vi "LoadSystemDefinition.vi"(8 "error in (no error)":errorcluster, 11 "SysDef.Path":path) -> (0 "error out":errorcluster, 2 "Aliases.Outputs":T1[](array[typedef]), 3 "Aliases.All":T1[](array[typedef]))   [LabVIEW 2015, in "Simple Sequence Tools - Editor.lvlib"]
uses:
  Simple Sequence Tools - Editor.lvlib
  Shared/Types/Channel.Properties.ctl
  NationalInstruments.VeriStand.SystemStorage
  NationalInstruments.VeriStand.SystemDefinitionAPI
  Shared/Simple Sequence Tools - Shared.lvlib
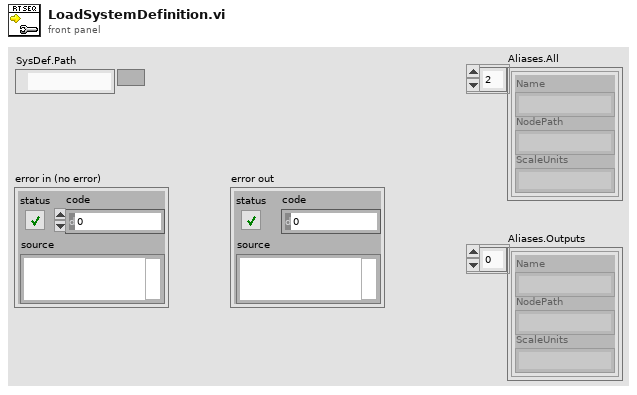
[diagram p1: front panel]
types:
  T1 = typedef "Simple Sequence Tools - Shared.lvlib/Channel.Properties.ctl" = cluster{"Name":string, "NodePath":string, "ScaleUnits":string}
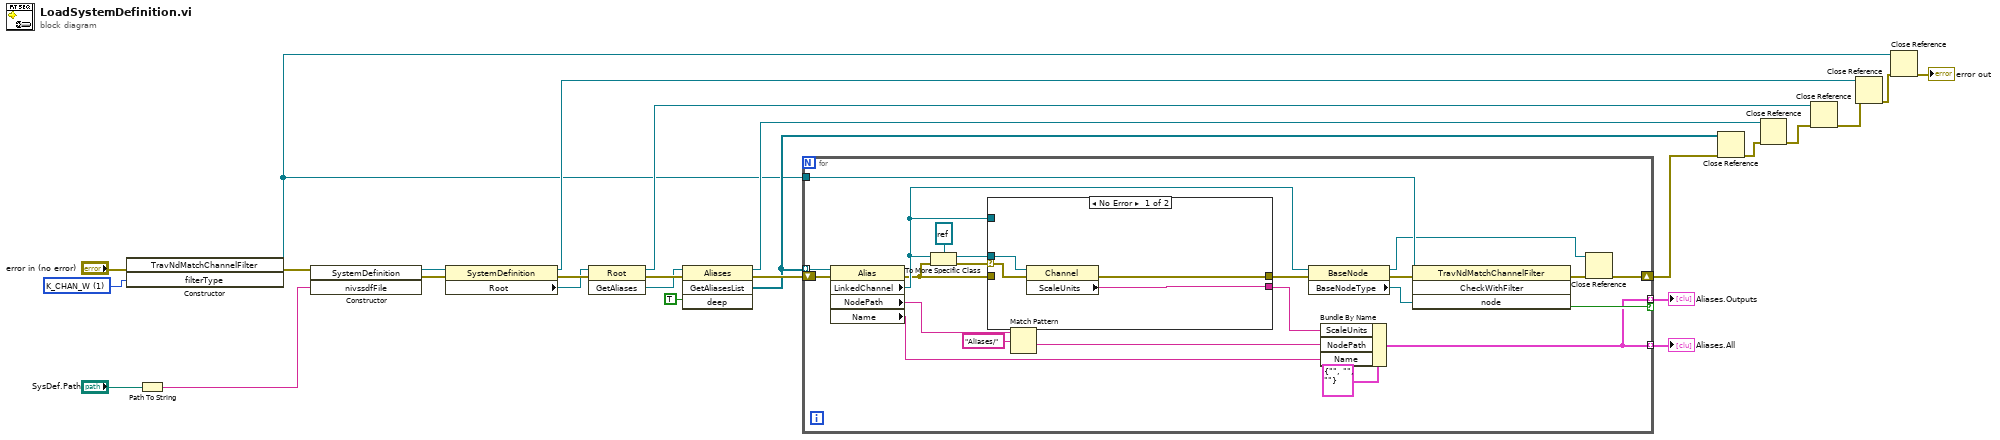
[diagram p0: block diagram]
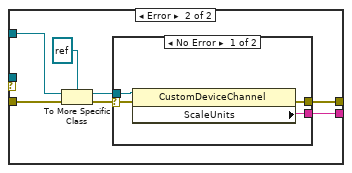
[diagram p2: hidden frame]
diagram:
  w16 = u8 1 items=["K_CHAN_R", "K_CHAN_W", "K_CHAN_VOLT", "K_CHAN_FAULT"] ("filterType")
  n1 = constructor class="TravNdMatchChannelFilter"(error in="error in (no error)", "filterType"=w16) -> (reference out=w9:refnum<k24>, error out=w14:errorcluster)  [unwired: 2 in, 2 out]
  n2 = Path To String(path="SysDef.Path") -> (string=w19:string)
  n3 = constructor class="SystemDefinition"(error in=w14, "nivssdfFile"=w19) -> (reference out=w20:refnum<k24>, error out=w25:errorcluster)  [unwired: 2 in, 2 out]
  n4 = property class="SystemDefinition"(reference=w20, error in=w25) -> (reference out=w13:refnum<k24>, error out=w24:errorcluster, "Root"=w21:refnum<k24>)
  n5 = invoke class="Root" method="GetAliases"(reference=w21, error in=w24) -> (reference out=w12:refnum<k24>, error out=w23:errorcluster, "GetAliases"=w17:refnum<k24>)  [unwired: 1 in]
  n6 = invoke class="Aliases" method="GetAliasesList"(reference=w17, error in=w23, "deep"=TRUE) -> (reference out=w11:refnum<k24>, error out=w26:errorcluster, "GetAliasesList"=w10:refnum<k24>[])  [unwired: 1 in, 1 out]
  n7 = for {
    tunnel: w10 -> [w48] mode=indexing
    tunnel: [w30] -> w2 mode=indexing if=w46
    shift-right: [w42] -> w4
    shift-left: w26 -> [w47]
    tunnel: [w30] -> w1 mode=indexing
    tunnel: w9 -> [w44]
    n8 = property class="Alias"(reference=w48, error in=w47) -> (error out=w37:errorcluster, "LinkedChannel"=w38:refnum<k24>, "NodePath"=w29:string, "Name"=w33:string)  [unwired: 1 out]
    n9 = To More Specific Class(target class=refnum<k24> refnum ("new reference"), reference=w38, error in=w37) -> (specific class reference=w40:refnum<k24>, error out=w41:errorcluster)
    n10 = case shown="No Error" w41 {
      selector: w41 -> [w51 _]
      tunnel: w40 -> [w52 _]
      tunnel: [w49 w54] -> w36
      tunnel: w38 -> [_ w59]
      tunnel: w37 -> [_ w58]
      tunnel: [w50 w53] -> w31
      frame No Error {
        n11 = property class="Channel"(reference=w52, error in=w51) -> (error out=w49:errorcluster, "ScaleUnits"=w50:string)  [unwired: 1 out]
      }
      frame Error {
        n12 = To More Specific Class(target class=refnum<k24> refnum ("new reference"), reference=w59, error in=w58) -> (specific class reference=w56:refnum<k24>, error out=w55:errorcluster)
        n13 = case shown="No Error" w55 {
          selector: w55 -> [w62 _]
          tunnel: w56 -> [w63 _]
          tunnel: [w61 _] -> w54
          tunnel: [w60 _] -> w53
          frame No Error {
            n14 = property class="CustomDeviceChannel"(reference=w63, error in=w62) -> (error out=w61:errorcluster, "ScaleUnits"=w60:string)  [unwired: 1 out]
          }
          frame Error {
          }
        }
      }
    }
    n15 = Match Pattern(string=w29, regular expression="Aliases/") -> (after substring=w28:string)  [unwired: 1 in, 3 out]
    n16 = property class="BaseNode"(reference=w38, error in=w36) -> (reference out=w35:refnum<k24>, error out=w45:errorcluster, "BaseNodeType"=w43:refnum<k24>)
    n17 = Bundle By Name(cluster=T1 {"Name"="", "NodePath"="", "ScaleUnits"=""}, "ScaleUnits"=w31, "NodePath"=w28, "Name"=w33) -> (w30:T1)
    n18 = invoke class="TravNdMatchChannelFilter" method="CheckWithFilter"(reference=w44, error in=w45, "node"=w43) -> (error out=w34:errorcluster, "CheckWithFilter"=w46:bool)  [unwired: 1 in, 2 out]
    n19 = Close Reference(reference=w35, error in (no error)=w34) -> (error out=w42:errorcluster)
  }
  "Aliases.Outputs" <- w2
  "Aliases.All" <- w1
  n20 = Close Reference(reference=w10, error in (no error)=w4) -> (error out=w8:errorcluster)
  n21 = Close Reference(reference=w11, error in (no error)=w8) -> (error out=w7:errorcluster)
  n22 = Close Reference(reference=w12, error in (no error)=w7) -> (error out=w6:errorcluster)
  n23 = Close Reference(reference=w13, error in (no error)=w6) -> (error out=w5:errorcluster)
  n24 = Close Reference(reference=w9, error in (no error)=w5) -> (error out=→"error out":errorcluster)
